vi "Ticks to Rotations (Drive).vi"(11 "Drive Velocities (ticks)":T1) -> (3 "Drive Velocities (rotations)":T1)   [LabVIEW 2023]
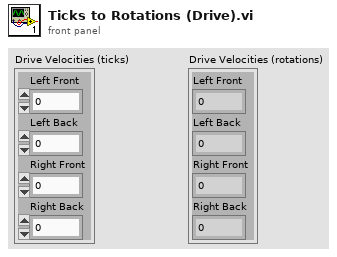
[diagram p1: front panel]
types:
  T1 = cluster{"Left Front":dbl, "Left Back":dbl, "Right Front":dbl, "Right Back":dbl}
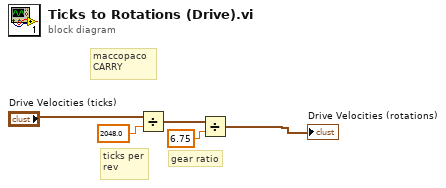
[diagram p0: block diagram]
diagram:
  # "ticks per\nrev"
  # "gear ratio"
  # "maccopaco\nCARRY"
  n1 = Divide(x="Drive Velocities (ticks)", y=2048.0) -> (x/y=w3:T1)
  n2 = Divide(x=w3, y=6.75) -> (x/y=→"Drive Velocities (rotations)":T1)
